vi "Host.vi"() -> ()   [LabVIEW 2025]
uses:
  <vilib>/rvi/interface/nirviOpenFPGA/nirviOpenFPGA.xnode
  <vilib>/rvi/interface/nirviMethod/nirviMethod.xnode
  <vilib>/FPGAPlugInAG/Dynamic/niLvFpga_Reset_Dynamic.vi
  <vilib>/rvi/interface/nirviCloseFPGA/nirviCloseFPGA.xnode
  <vilib>/FPGAPlugInAG/Dynamic/niLvFpga_Run_Dynamic.vi
  <vilib>/rvi/errors/niLvFpgaMergeErrorWithErrorCode.vi
  <vilib>/FPGAPlugInAG/Dynamic/niLvFpga_ReadFifo_Dynamic.vi
  Paper-Online-FPGA/V1.0/FPGA Bitfiles/project_FPGATarget_128-32-16-8-2_YG1qj7JyXO8.lvbitx
  Paper-Online-FPGA/V1.0/128-32-16-8-2.vi
  <vilib>/FPGAPlugInAG/cRIO-9033/niLvFpga_Open_cRIO-9033.vi
  <vilib>/rvi/interface/common/dynamic/niFpgaDynamicAddResources.vi
  <vilib>/FPGAPlugInAG/Dynamic/niLvFpga_WriteFifo_Dynamic.vi
  <vilib>/FPGAPlugInAG/Dynamic/niLvFpga_Close_Dynamic.vi
panel:
  out "Window(s)":dbl[](array[numeric])
  out "input":dbl[](array[numeric])
  out "size(s)":i32
  out "Timing":fxp<+,32,16>[](array[numeric])
  out "Healthy%":fxp<+,34,2>[](array[numeric])
  out "Unhealthy%":fxp<+/-,33,1>[](array[numeric])
  out "Uncontrolled Acceleration":dynamicdata(graph)
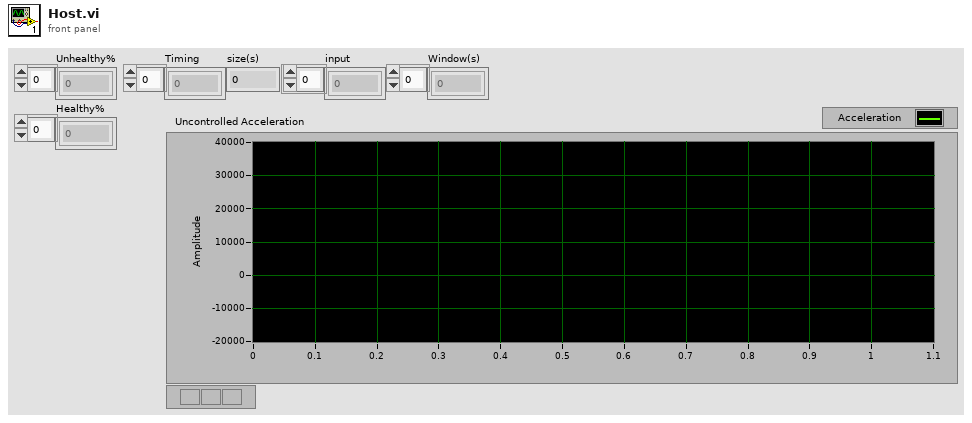
[diagram p1: front panel]
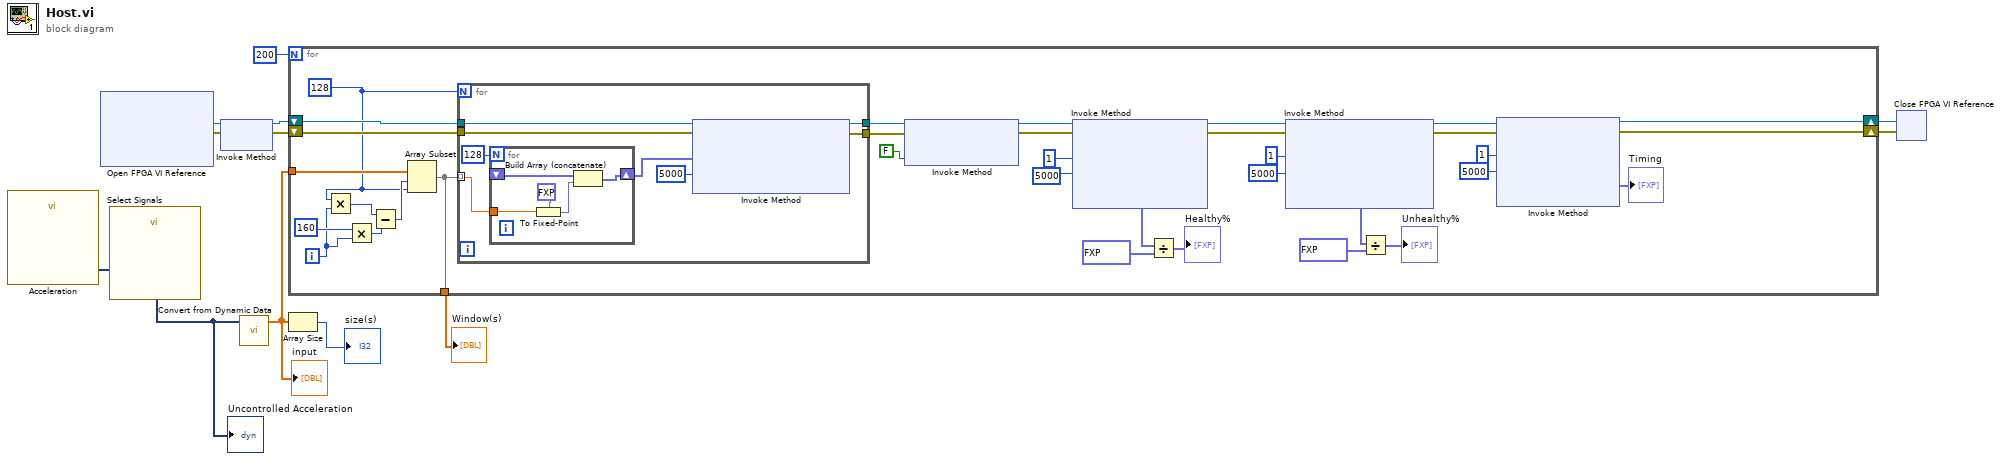
[diagram p0: block diagram]
diagram:
  n1 = call "Acceleration"() -> ("Signals"=w12:dynamicdata)  [unwired: 6 in, 5 out]
  n2 = xnode "Open FPGA VI Reference"() -> ("FPGA VI Reference Out"=w11:refnum<k20>, "error out"=w8:errorcluster)  [unwired: 2 in]
  n3 = call "Select Signals"("Signals"=w12) -> ("Signal Out"=w7:dynamicdata)  [unwired: 9 in, 1 out]
  "Uncontrolled Acceleration" <- w7
  n4 = xnode "Invoke Method"("FPGA VI Reference In"=w11, "error in"=w8) -> ("FPGA VI Reference Out"=w10:refnum<k20>, "error out"=w9:errorcluster)
  n5 = call "Convert from Dynamic Data"("Dynamic Data Type"=w7) -> ("Array"=w2:dbl[])  [unwired: 3 in]
  "input" <- w2
  n6 = for {
    N: 200 -> [_]
    shift-right: [w28] -> w6
    shift-left: w10 -> [w46]
    shift-right: [w27] -> w5
    shift-left: w9 -> [w45]
    tunnel: w2 -> [w39]
    tunnel: [w24] -> w1
    i -> [w35]
    w33 = 128
    n7 = Multiply(x=w33, y=w35) -> (x*y=w38:i32)
    n8 = Multiply(x=160 ("y"), y=w35) -> (x*y=w34:i32)
    n9 = Subtract(x=w38, y=w34) -> (x-y=w37:i32)
    n10 = Array Subset(array=w39, index=w37, length=w33) -> (w24:dbl[])
    n11 = for {
      N: w33 -> [_]
      tunnel: w46 -> [w54]
      tunnel: w45 -> [w53]
      tunnel: [w52] -> w41
      tunnel: [w51] -> w40
      tunnel: w24 -> [w48] mode=indexing
      n12 = for {
        N: 128 -> [_]
        tunnel: w48 -> [w58]
        shift-right: [w56] -> w47
        shift-left: _ -> [w55]
        n13 = To Fixed-Point(fixed-point type=fxp<+/-,32,16> 0.0, number=w58) -> (fixed-point=w57:fxp<+/-,32,16>)
        n14 = Build Array (concatenate)(w55, w57) -> (w56:fxp<+/-,32,16>[])
      }
      n15 = xnode "Invoke Method"("FPGA VI Reference In"=w54, "error in"=w53, "Data"=w47, "Timeout (ms)"=5000) -> ("FPGA VI Reference Out"=w52:refnum<k20>, "error out"=w51:errorcluster)  [unwired: 1 out]
    }
    n16 = xnode "Invoke Method"("FPGA VI Reference In"=w41, "error in"=w40, "Wait Until Done (F)"=FALSE) -> ("FPGA VI Reference Out"=w43:refnum<k20>, "error out"=w42:errorcluster)
    n17 = xnode "Invoke Method"("FPGA VI Reference In"=w43, "error in"=w42, "Number of Elements"=u32 1, "Timeout (ms)"=5000) -> ("FPGA VI Reference Out"=w32:refnum<k20>, "error out"=w31:errorcluster, "Data"=w20:fxp<+,33,17>[])  [unwired: 1 out]
    n18 = Divide(x=w20, y=fxp<+,1,16>[] [32768.0]) -> (x/y=→"Healthy%":fxp<+,34,2>[])
    n19 = xnode "Invoke Method"("FPGA VI Reference In"=w32, "error in"=w31, "Number of Elements"=u32 1, "Timeout (ms)"=5000) -> ("FPGA VI Reference Out"=w26:refnum<k20>, "error out"=w25:errorcluster, "Data"=w23:fxp<+/-,32,16>[])  [unwired: 1 out]
    n20 = Divide(x=w23, y=fxp<+,1,16>[] [32768.0]) -> (x/y=→"Unhealthy%":fxp<+/-,33,1>[])
    n21 = xnode "Invoke Method"("FPGA VI Reference In"=w26, "error in"=w25, "Number of Elements"=u32 1, "Timeout (ms)"=5000) -> ("FPGA VI Reference Out"=w28:refnum<k20>, "error out"=w27:errorcluster, "Data"=→"Timing":fxp<+,32,16>[])  [unwired: 1 out]
  }
  "Window(s)" <- w1
  n22 = Array Size(array=w2) -> (size(s)=→"size(s)":i32)
  n23 = xnode "Close FPGA VI Reference"("FPGA VI Reference In"=w6, "error in"=w5) -> ()  [unwired: 1 out]
